vi "Set TestData.vi"(8 "error in (no error)":errorcluster, 11 "Main":refnum<vi>) -> (0 "error out":errorcluster, 2 "dS":dbl, 3 "XY Plot out":refnum<vi>)   [LabVIEW 2025, in "Flow Grind.lvlib" / "4way Lap.lvclass"]
uses:
  4way Lap.lvclass
  <vilib>/Analysis/6fits.llb/Curve Fitting Criteria.ctl
  1fd75abc-c2ef-4fe7-a3c8-a47552fa74cb.vi
  <vilib>/Array/Sort 2D Array - Pop Stack.vi
  <vilib>/Array/Sort 2D Array - Push Stack.vi
  1fd75abc-c2ef-4fe7-a3c8-a47552fa74cb.vi/269d4b3b-47f5-49e3-8884-44851e4dd9d5.vi
  1fd75abc-c2ef-4fe7-a3c8-a47552fa74cb.vi/6d99389c-673d-4efb-bf33-19b32bcf4cf8.vi
  <vilib>/Analysis/NI_AALPro.lvlib
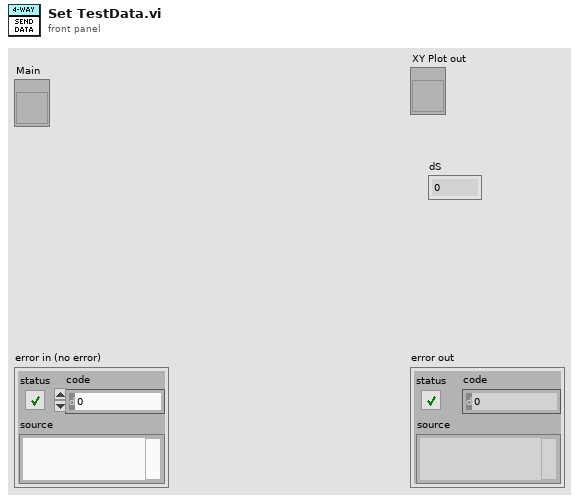
[diagram p1: front panel]
types:
  T1 = typedef "NI_AALPro.lvlib/Curve Fitting Criteria.ctl" = u16
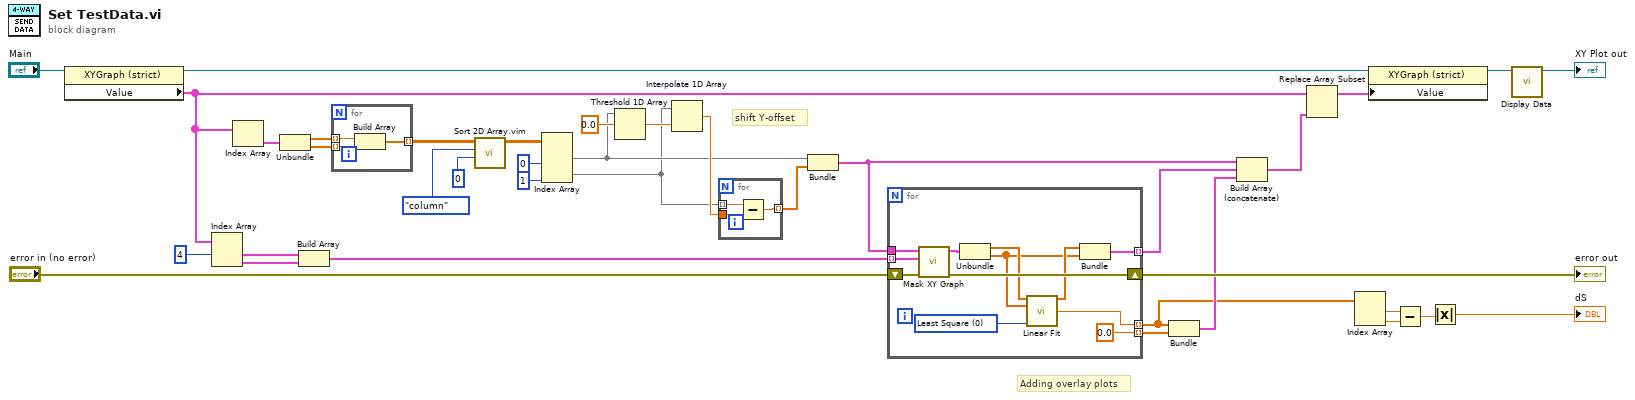
[diagram p0: block diagram]
diagram:
  # "Adding overlay plots"
  # "shift Y-offset"
  n1 = property class="XYGraph (strict)"(reference="Main") -> (reference out=w11:refnum<vi>, "Value"=w9:cluster{dbl[], dbl[]}[])  [unwired: 1 in, 1 out]
  n2 = Index Array(array=w9, index #1=4 ("index")) -> (element #1=w14:cluster{dbl[], dbl[]}, element #2=w13:cluster{dbl[], dbl[]})  [unwired: 1 in]
  n3 = Index Array(array=w9) -> (element=w18:cluster{dbl[], dbl[]})  [unwired: 1 in]
  n4 = Unbundle(w18) -> (w17:dbl[], w31:dbl[])
  n5 = Build Array(w14, w13) -> (w12:cluster{dbl[], dbl[]}[])
  n6 = for {
    tunnel: w17 -> [w40] mode=indexing
    tunnel: w31 -> [w39] mode=indexing
    tunnel: [w38] -> w32 mode=indexing
    n7 = Build Array(w40, w39) -> (w38:dbl[])
  }
  n8 = call "Sort 2D Array.vim"("index"=0, "dimension to index (column)"=enum16{"column", "row"}."column", "2D array"=w32) -> ("sorted 2D array"=w35:dbl[][])  [unwired: 7 in, 1 out]
  n9 = Index Array(array=w35, index (col) #1=0 ("index (row)"), index (col) #2=1 ("index (col)")) -> (element #1=w26:dbl[], element #2=w25:dbl[])  [unwired: 2 in]
  n10 = Threshold 1D Array(2:0.0 ("fractional index or x"), 3:w26) -> (0:w28:dbl)  [unwired: 1 in]
  n11 = Interpolate 1D Array(1:w28, 2:w25) -> (0:w37:dbl)
  n12 = for {
    tunnel: w37 -> [w42]
    tunnel: [w43] -> w27 mode=indexing
    tunnel: w25 -> [w41] mode=indexing
    n13 = Subtract(x=w41, y=w42) -> (x-y=w43:dbl)
  }
  n14 = Bundle("sorted 2D array"=w26, w27) -> (w20:cluster{"sorted 2D array":dbl[], dbl[]})  [unwired: 1 in]
  n15 = for {
    tunnel: w20 -> [w55]
    tunnel: w12 -> [w54] mode=indexing
    shift-right: [w52] -> w23
    shift-left: "error in (no error)" -> [w53]
    tunnel: [w50] -> w22 mode=indexing
    tunnel: [w44] -> w1 mode=indexing
    tunnel: [0.0 ("fractional index or x")] -> w19 mode=indexing
    w48 = T1 0 items=["Least Square", "Least Absolute Residual", "Bisquare"] ("method")
    n16 = call "Mask XY Graph.vi"("error in (no error)"=w53, "Mask"=w54, "Data"=w55) -> ("error out"=w52:errorcluster, "Masked Data"=w51:cluster{"X":dbl[], "Y":dbl[]})  [unwired: 6 in, 1 out]
    n17 = Unbundle(w51) -> ("X"=w47:dbl[], "Y"=w45:dbl[])
    n18 = call <vilib>:"Linear Fit.vi"("Y"=w47, "X"=w45, "method"=w48) -> ("Best Linear Fit"=w46:dbl[], "intercept"=w44:dbl)  [unwired: 8 in, 3 out]
    n19 = Bundle("Best Linear Fit"=w46, "Y"=w45) -> (w50:cluster{"Best Linear Fit":dbl[], "Y":dbl[]})  [unwired: 1 in]
  }
  "error out" <- w23
  n20 = Bundle(w1, w19) -> (w21:cluster{dbl[], dbl[]})  [unwired: 1 in]
  n21 = Build Array (concatenate)(w20, w22, w21) -> (w8:cluster{"Best Linear Fit":dbl[], "Y":dbl[]}[])
  n22 = Replace Array Subset(array=w9, new element=w8) -> (w7:cluster{dbl[], dbl[]}[])  [unwired: 1 in]
  n23 = Index Array(array=w1) -> (element #1=w4:dbl, element #2=w2:dbl)  [unwired: 2 in]
  n24 = property class="XYGraph (strict)"(reference=w11, "Value"=w7) -> (reference out=w10:refnum<vi>)  [unwired: 1 in, 1 out]
  n25 = Subtract(x=w4, y=w2) -> (x-y=w3:dbl)
  n26 = Absolute Value(x=w3) -> (abs(x)=→"dS":dbl)
  n27 = call "Display Data.vi"("XY Plot"=w10) -> ("XY Plot out"=→"XY Plot out":refnum<vi>)  [unwired: 9 in, 1 out]
